vi "_FormatText.vi"(7 "TextSettings":T1={"Desired Font"="Application Font", "Strikeout?"=FALSE, "Italic?"=FALSE, "Underline?"=FALSE, "Outline?"=FALSE, "Shadow?"=FALSE, "Bold?"=FALSE, "Size"=12}, 9 "Angle":dbl, 10 "MaxLength":i32, 11 "Text":string) -> (2 "NewHeight":i32, 3 "FormatedText":string)   [LabVIEW 2020, in "OpenLvVision_Overlays.lvlib"]
uses:
  OpenLvVision_Overlays.lvlib
  TypeDefs/TextSettings.ctl
  <vilib>/Utility/error.llb/whitespace.ctl
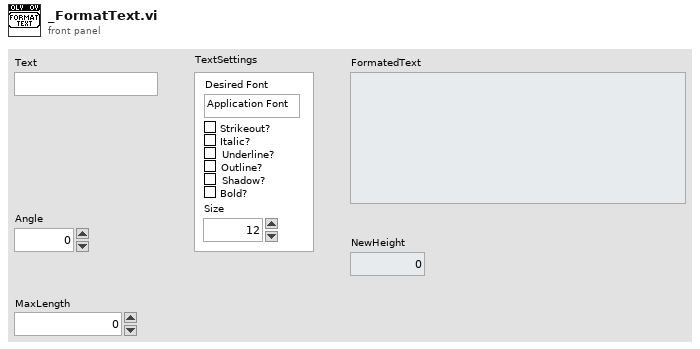
[diagram p1: front panel]
types:
  T1 = typedef "OpenLvVision_Overlays.lvlib/TextSettings.ctl" = cluster{"Desired Font":string, "Strikeout?":bool, "Italic?":bool, "Underline?":bool, "Outline?":bool, "Shadow?":bool, "Bold?":bool, "Size":i32}
  T2 = typedef "whitespace.ctl" = u16
  T3 = cluster{"horizontal":enum16{"left", "center", "right"}, "vertical":enum16{"top", "center", "bottom"}}
  T4 = enum16{"User-specified Font", "Application Font", "System Font", "Dialog Font"}
  T5 = cluster{"Font Name:":string, "Size":i16, "Strikeout?":bool, "Italic?":bool, "Underline?":bool, "Outline?":bool, "Shadow?":bool, "Bold?":bool}
  T6 = cluster{"left":i16, "top":i16, "right":i16, "bottom":i16}
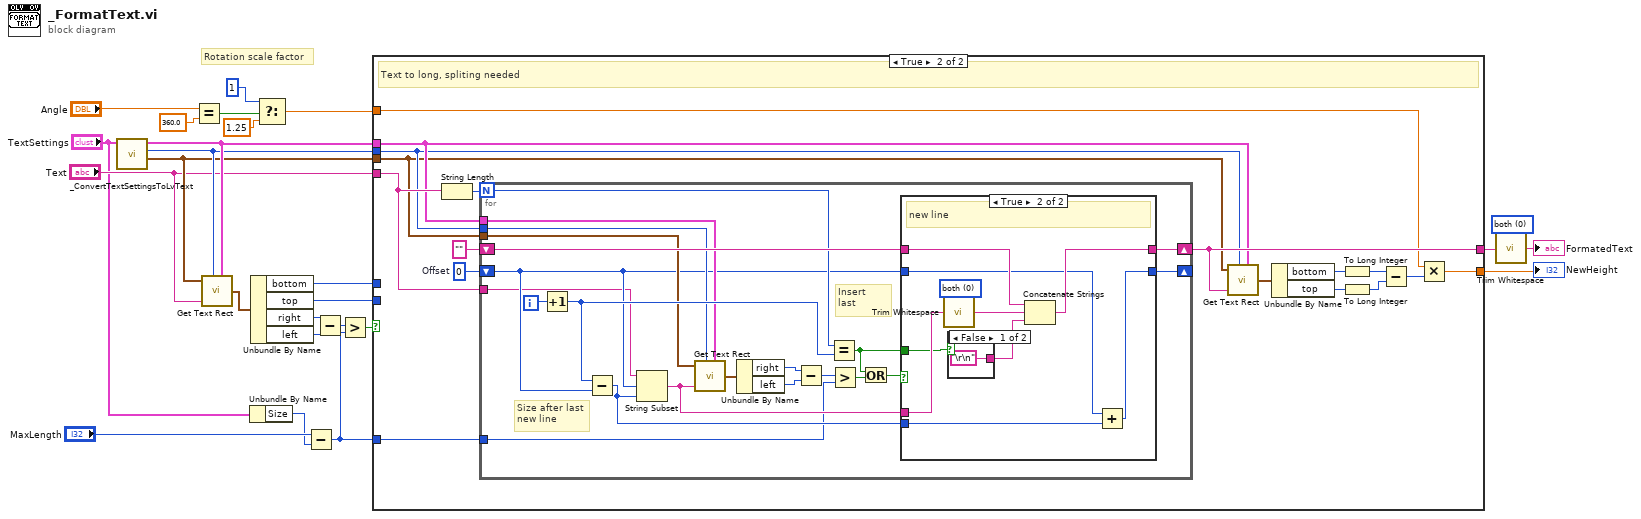
[diagram p0: block diagram]
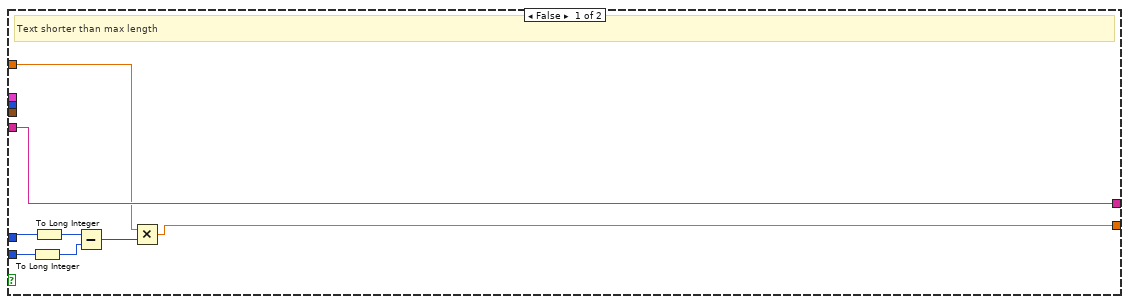
[diagram p2: hidden frame]
diagram:
  w1 = T2 0 items=["both", "start of string", "end of string"] ("location (both)")
  # "Rotation scale factor"
  n1 = call "_ConvertTextSettingsToLvText.vi"("TextSettings"="TextSettings") -> ("alignment"=w20:T3, "desired font"=w21:T4, "[user-specified font]"=w22:T5)  [unwired: 8 in]
  n2 = Equal?(x="Angle", y=360.0) -> (x = y?=w12:bool)
  n3 = call <vilib>:"Get Text Rect.vi"("alignment(left, top)"=w20, "desired font(Application)"=w21, "text"="Text", "[user-specified font]"=w22) -> ("rect"=w25:T6)  [unwired: 5 in]
  n4 = Unbundle By Name("TextSettings") -> ("Size"=w6:i32)
  n5 = Unbundle By Name(w25) -> ("bottom"=w17:i16, "top"=w16:i16, "right"=w4:i16, "left"=w5:i16)
  n6 = Select(t=1, s=w12, f=1.25) -> (s? t:f=w10:dbl)
  n7 = Subtract(x="MaxLength", y=w6) -> (x-y=w8:i32)
  n8 = Subtract(x=w4, y=w5) -> (x-y=w24:i16)
  n9 = Greater?(x=w24, y=w8) -> (0:w23:bool)
  n10 = case shown="True" w23 {
    tunnel: w22 -> [_ w43]
    tunnel: w21 -> [_ w42]
    tunnel: w20 -> [_ w41]
    tunnel: "Text" -> [w33 w44]
    tunnel: w8 -> [_ w49]
    tunnel: [w33 w45] -> w3
    tunnel: [w27 w35] -> w18
    tunnel: w17 -> [w32 _]
    tunnel: w16 -> [w31 _]
    tunnel: w10 -> [w26 w34]
    frame False {
      # "Text shorter than max length"
      n11 = To Long Integer(number=w31) -> (32bit integer=w29:i32)
      n12 = To Long Integer(number=w32) -> (32bit integer=w30:i32)
      n13 = Subtract(x=w30, y=w29) -> (x-y=w28:i32)
      n14 = Multiply(x=w26, y=w28) -> (x*y=w27:dbl)
    }
    frame True {
      w47 = 0  # Offset
      # "Text to long, spliting needed"
      n15 = String Length(string=w44) -> (length=w50:i32)
      n16 = for {
        N: w50 -> [w58]
        tunnel: w41 -> [w54]
        tunnel: w42 -> [w56]
        tunnel: w43 -> [w55]
        tunnel: w49 -> [w61]
        shift-right: [w71] -> w45
        shift-left: "" -> [w70]
        shift-right: [w69] -> _
        shift-left: w47 -> [w53]
        tunnel: w44 -> [w52]
        i -> [w64]
        # "Insert\nlast"
        # "Size after last \nnew line"
        n17 = Increment(x=w64) -> (x+1=w57:i32)
        n18 = Subtract(x=w57, y=w53) -> (x-y=w62:i32)
        n19 = String Subset(string=w52, offset (0)=w53, length (rest)=w62) -> (substring=w63:string)
        n20 = call <vilib>:"Get Text Rect.vi"("alignment(left, top)"=w54, "desired font(Application)"=w56, "text"=w63, "[user-specified font]"=w55) -> ("rect"=w65:T6)  [unwired: 5 in]
        n21 = Unbundle By Name(w65) -> ("right"=w67:i16, "left"=w66:i16)
        n22 = Subtract(x=w67, y=w66) -> (x-y=w68:i16)
        n23 = Equal?(x=w58, y=w57) -> (x = y?=w51:bool)
        n24 = Greater?(x=w68, y=w61) -> (0:w59:bool)
        n25 = Or(x=w51, y=w59) -> (x .or. y?=w60:bool)
        n26 = case shown="True" w60 {
          tunnel: [w73 w82] -> w71
          tunnel: w70 -> [w73 w83]
          tunnel: [w72 w78] -> w69
          tunnel: w53 -> [w72 w79]
          tunnel: w63 -> [_ w75]
          tunnel: w62 -> [_ w77]
          tunnel: w51 -> [_ w74]
          frame False {
          }
          frame True {
            w80 = T2 0 items=["both", "start of string", "end of string"] ("location (both)")
            # "new line"
            n27 = call <vilib>:"Trim Whitespace.vi"("string"=w75, "location (both)"=w80) -> ("trimmed string"=w81:string)
            n28 = case shown="False" w74 {
              tunnel: ["\r\n" _] -> w76
              frame False {
              }
              frame True {
              }
            }
            n29 = Concatenate Strings(w83, w81, w76) -> (w82:string)
            n30 = Add(x=w79, y=w77) -> (x+y=w78:i32)
          }
        }
      }
      n31 = call <vilib>:"Get Text Rect.vi"("alignment(left, top)"=w41, "desired font(Application)"=w42, "text"=w45, "[user-specified font]"=w43) -> ("rect"=w46:T6)  [unwired: 5 in]
      n32 = Unbundle By Name(w46) -> ("bottom"=w40:i16, "top"=w39:i16)
      n33 = To Long Integer(number=w40) -> (32bit integer=w38:i32)
      n34 = To Long Integer(number=w39) -> (32bit integer=w37:i32)
      n35 = Subtract(x=w38, y=w37) -> (x-y=w36:i32)
      n36 = Multiply(x=w34, y=w36) -> (x*y=w35:dbl)
    }
  }
  "NewHeight" <- w18
  n37 = call <vilib>:"Trim Whitespace.vi"("string"=w3, "location (both)"=w1) -> ("trimmed string"=→"FormatedText":string)
